vi "Latency Add.vi"(10 "value (us)":dbl, 11 "metric in":T1) -> (3 "metric out":T1)   [LabVIEW 2021, in "CAN_Reader_CANsub_Test_Helpers.lvlib"]
uses:
  CAN_Reader_CANsub_Test_Helpers.lvlib
  Latency Metric.ctl
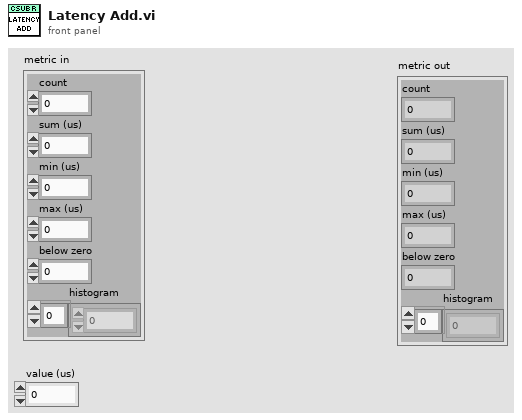
[diagram p1: front panel]
types:
  T1 = typedef "CAN_Reader_CANsub_Test_Helpers.lvlib/Latency Metric.ctl" = cluster{"count":u32, "sum (us)":dbl, "min (us)":dbl, "max (us)":dbl, "below zero":u32, "histogram":u32[]}
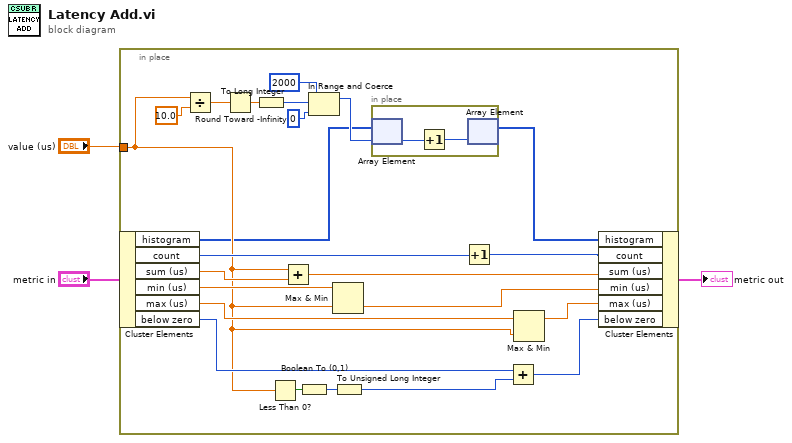
[diagram p0: block diagram]
diagram:
  n1 = in-place {
    in-place-border: "value (us)" -> [w7]
    n2 = in-place-cluster #1("metric in") -> ("histogram"=w5:u32[], "count"=w26:u32, "sum (us)"=w24:dbl, "min (us)"=w22:dbl, "max (us)"=w20:dbl, "below zero"=w16:u32)
    n3 = Divide(x=w7, y=10.0) -> (x/y=w13:dbl)
    n4 = Round Toward -Infinity(1:w13) -> (0:w12:dbl)
    n5 = To Long Integer(number=w12) -> (32bit integer=w11:i32)
    n6 = Less Than 0?(x=w7) -> (x < 0?=w18:bool)
    n7 = Add(x=w7, y=w24) -> (x+y=w23:dbl)
    n8 = Boolean To (0,1)(Boolean=w18) -> (0, 1=w17:i16)
    n9 = In Range and Coerce(upper limit=2000, x=w11, lower limit=0) -> (coerced(x)=w6:i32)  [unwired: 1 out]
    n10 = Max & Min(x=w22, y=w7) -> (min(x,y)=w21:dbl)  [unwired: 1 out]
    n11 = To Unsigned Long Integer(number=w17) -> (unsigned 32bit integer=w15:u32)
    n12 = in-place {
      n13 = in-place-array #2(w5, w6) -> (w28:u32)
      n14 = Increment(x=w28) -> (x+1=w27:u32)
      n15 = in-place-array #2(w27) -> (w4:u32[])  [unwired: 1 out]
    }
    n16 = Increment(x=w26) -> (x+1=w25:u32)
    n17 = Add(x=w16, y=w15) -> (x+y=w14:u32)
    n18 = Max & Min(x=w20, y=w7) -> (max(x,y)=w19:dbl)  [unwired: 1 out]
    n19 = in-place-cluster #1("histogram"=w4, "count"=w25, "sum (us)"=w23, "min (us)"=w21, "max (us)"=w19, "below zero"=w14) -> (→"metric out":T1)
  }
